vi "Remote Run.vi"() -> ()   [LabVIEW 2020]
doc: "Dev helper: runs a VI in another LabVIEW over VI Server (machine, port; e.g. LabVIEW 2020 on 3365 next to LabVIEW 2026) and waits for it. inputs sets controls first: per element the control name and its value as LabVIEW XML wrapped in LvVariant (the type travels with it, so a path, a number or a cluster can be set). After the run the control named result is read and returned as LabVIEW XML. The VI must not be running there already."
panel:
  out "error out":errorcluster
  out "result xml":string
  in  "result":string="error out"
  in  "inputs":cluster{"name":string, "xml":string}[](array[cluster])
  in  "vi path":path
  in  "port":u32=3365
  in  "machine":string="localhost"
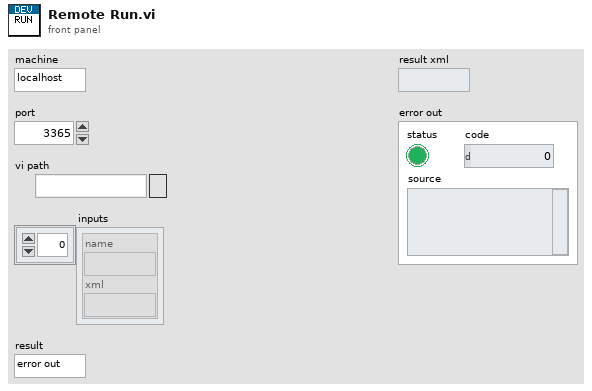
[diagram p1: front panel]
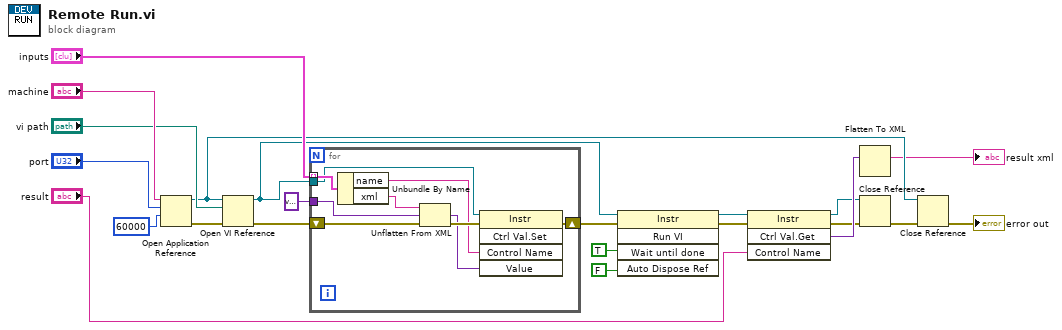
[diagram p0: block diagram]
diagram:
  n1 = Open Application Reference(9:60000, 10:"port", 11:"machine") -> (0:w18:errorcluster, 3:w4:refnum<vi>)  [unwired: 1 in]
  n2 = Open VI Reference(application reference (local)=w4, vi path="vi path", error in (no error)=w18) -> (vi reference=w14:refnum<vi>, error out=w15:errorcluster)  [unwired: 3 in]
  n3 = for {
    tunnel: "inputs" -> [w31] mode=indexing
    tunnel: w14 -> [w27]
    tunnel: variant -> [w29]
    shift-right: [w23] -> w13
    shift-left: w15 -> [w28]
    n4 = Unbundle By Name(w31) -> ("name"=w25:string, "xml"=w30:string)
    n5 = Unflatten From XML(xml string=w30, type=w29, error in (no error)=w28) -> (value=w24:variant, error out=w26:errorcluster)
    n6 = invoke class="Instr" method="Ctrl Val.Set"(reference=w27, error in=w26, "Control Name"=w25, "Value"=w24) -> (error out=w23:errorcluster)  [unwired: 1 in, 4 out]
  }
  n7 = invoke class="Instr" method="Run VI"(reference=w14, error in=w13, "Wait until done"=TRUE, "Auto Dispose Ref"=FALSE) -> (reference out=w10:refnum<vi>, error out=w9:errorcluster)  [unwired: 1 in, 3 out]
  n8 = invoke class="Instr" method="Ctrl Val.Get"(reference=w10, error in=w9, "Control Name"="result") -> (reference out=w6:refnum<vi>, error out=w5:errorcluster, "Get Control Value Variant"=w7:variant)  [unwired: 1 in, 1 out]
  n9 = Flatten To XML(6:w7) -> (2:→"result xml":string)
  n10 = Close Reference(reference=w6, error in (no error)=w5) -> (error out=w3:errorcluster)
  n11 = Close Reference(reference=w4, error in (no error)=w3) -> (error out=→"error out":errorcluster)
